vi "Register for Broadcasting Events Recursively.vi"(8 "error in (no error)":errorcluster, 10 "Event Registration Refnum In":refnum<event-registration>, 11 "Application In":refnum<class "Application.lvclass">) -> (0 "error out":errorcluster, 2 "Event Registration Refnum Out":refnum<event-registration>, 3 "Application Out":refnum<class "Application.lvclass">)   [LabVIEW 2020, in "Application.lvclass"]
doc: "Register for the broad cast events for the application and nested processes."
uses:
  Application.lvclass
  Process/Protected/Broadcasting/Broadcast Message Cluster.ctl
  Application.lvclass/Application.ctl
  Process/Process.lvclass
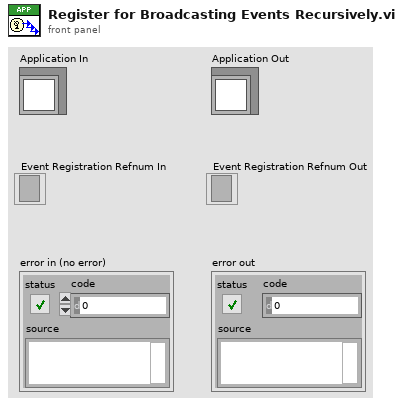
[diagram p1: front panel]
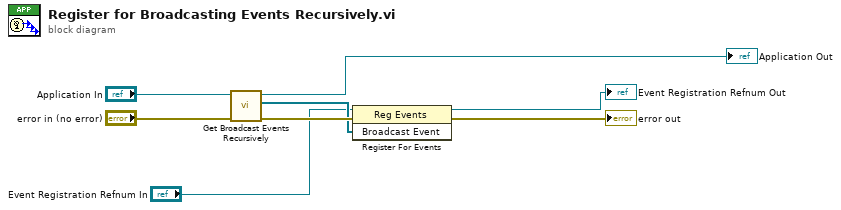
[diagram p0: block diagram]
diagram:
  n1 = call "Get Broadcast Events Recursively.vi"("error in (no error)"="error in (no error)", "Application In"="Application In") -> ("error out"=w7:errorcluster, "Broadcast Event"=w6:refnum<user-event>[], "Application Out"=→"Application Out":refnum<class "Application.lvclass">)  [unwired: 7 in]
  n2 = register-events(reference="Event Registration Refnum In", error in=w7, w6) -> (reference out=→"Event Registration Refnum Out":refnum<event-registration>, error out=→"error out":errorcluster)
